vi "FOR.vi"() -> ()   [LabVIEW 2026]
panel:
  out "NÚMEROS GENERADOS":dbl[](array[numeric])
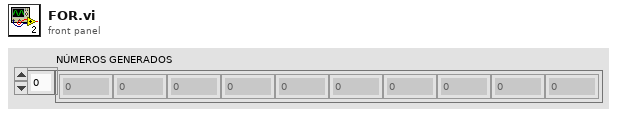
[diagram p1: front panel]
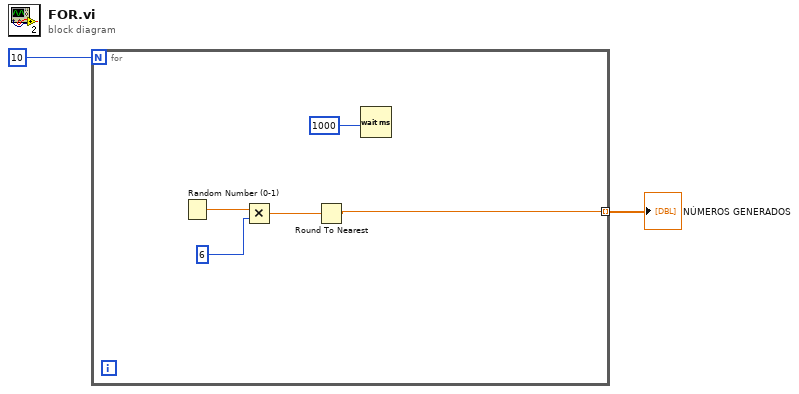
[diagram p0: block diagram]
diagram:
  n1 = for {
    N: 10 -> [_]
    tunnel: [w3] -> w2 mode=indexing
    n2 = Random Number (0-1)() -> (number: 0 to 1=w7:dbl)
    n3 = Multiply(x=w7, y=6) -> (x*y=w4:dbl)
    n4 = Round To Nearest(number=w4) -> (nearest integer value=w3:dbl)
    n5 = Wait (ms)(milliseconds to wait=1000) -> ()  [unwired: 1 out]
  }
  "NÚMEROS GENERADOS" <- w2
